vi "validate.vi"(8 "error in":errorcluster, 11 "configuration in":refnum<class "PL_System Configuration.lvclass">) -> (0 "error out":errorcluster, 3 "configuration out":refnum<class "PL_System Configuration.lvclass">)   [LabVIEW 2013, in "PL_System Configuration.lvclass"]
doc: "Provides an interface for performing validation on a given configuration. Any children should define the behavior of this function to ensure that the configuration in memory can be used by the runtime class."
uses:
  PL_System Configuration.lvclass
  <vilib>/NI/Tag Bus Module Framework/root configuration/TBM configuration.lvclass
  <vilib>/NI/Configuration Framework/serializable configuration/get alias.vi
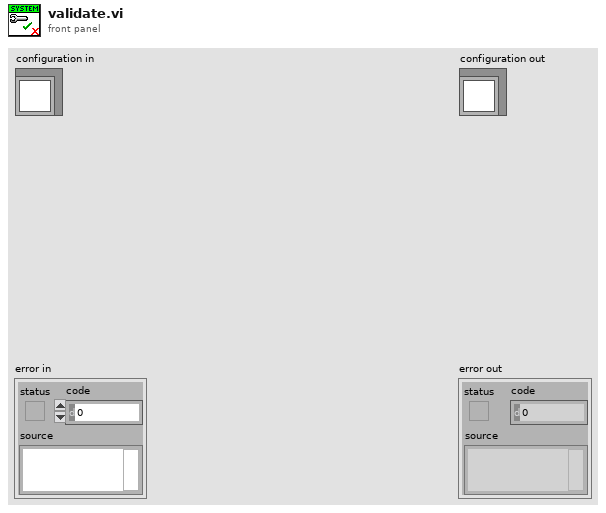
[diagram p1: front panel]
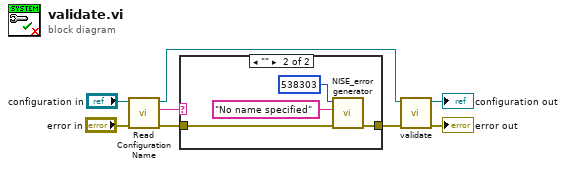
[diagram p0: block diagram]
diagram:
  n1 = call "Read Configuration Name.vi"("error in"="error in", "PL_System Configuration in"="configuration in") -> ("error out"=w4:errorcluster, "Configuration Name"=w1:string, "PL_System Configuration out"=w2:refnum<class "PL_System Configuration.lvclass">)  [unwired: 7 in]
  n2 = case shown="\"\"" w1 {
    tunnel: [w9 w12] -> w6
    tunnel: w4 -> [w9 w13]
    frame Default {
    }
    frame "" {
      n3 = call <vilib>:"NISE_error generator.vi"("error in"=w13, "append error message"="No name specified" ("error message (\"\")"), "error code (0)"=538303) -> ("error out"=w12:errorcluster)  [unwired: 6 in]
    }
  }
  n4 = call-parent "validate.vi"("error in"=w6, "configuration in"=w2) -> ("error out"=→"error out":errorcluster, "configuration out"=→"configuration out":refnum<class "PL_System Configuration.lvclass">)  [unwired: 8 in]
